vi "Test Assert Equal Value (Typedef).vi"(8 "error in":errorcluster) -> (0 "error out":errorcluster)   [LabVIEW 2020]
uses:
  <vilib>/Utility/error.llb/ErrWarn.ctl
  <vilib>/Utility/error.llb/DialogTypeEnum.ctl
  <vilib>/picture/picture.llb/imagedata.ctl
  <vilib>/Utility/miscctls.llb/LVBoundsTypeDef.ctl
  classes/Assert/Assert Equal Value_Variant.vi
  classes/Assert/Assert.lvclass
  classes/Test/Test.lvclass
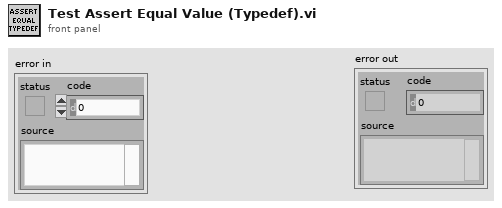
[diagram p1: front panel]
types:
  T1 = typedef "LVBoundsTypeDef.ctl" = cluster{"Width":u32, "Height":u32}
  T2 = cluster{"image type":i32, "image depth":i32, "image":u8[], "mask":u8[], "colors":u32[], "Rectangle":cluster{"left":i16, "top":i16, "right":i16, "bottom":i16}}
  T3 = typedef "imagedata.ctl" = cluster{"image type":i32, "image depth":i32, "image":u8[], "mask":u8[], "colors":u32[], "Rectangle":cluster{"left":i16, "top":i16, "right":i16, "bottom":i16}}
  T4 = enum16{"no dialog", "OK message", "continue or stop message", "auto error handling dialog", "OK message + warnings", "continue/stop + warnings"}
  T5 = typedef "DialogTypeEnum.ctl" = enum16{"no dialog", "OK message", "continue or stop message", "auto error handling dialog", "OK message + warnings", "continue/stop + warnings"}
  T6 = typedef "ErrWarn.ctl" = bool
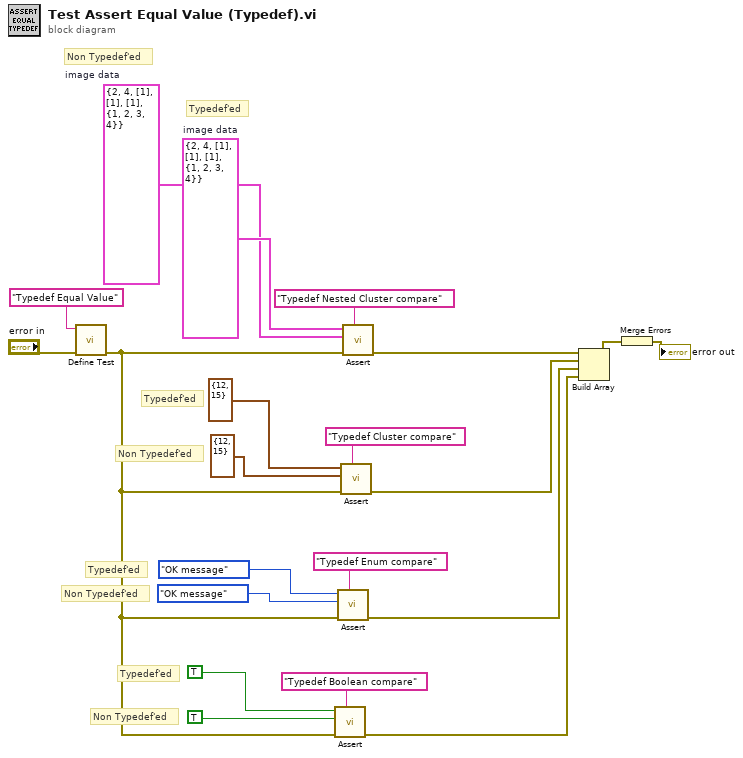
[diagram p0: block diagram]
diagram:
  w14 = T2 {"image type"=2, "image depth"=4, "image"=[1], "mask"=[1], "colors"=[1], "Rectangle"={"left"=1, "top"=2, "right"=3, "bottom"=4}}  # image data
  w15 = T3 {"image type"=2, "image depth"=4, "image"=[1], "mask"=[1], "colors"=[1], "Rectangle"={"left"=1, "top"=2, "right"=3, "bottom"=4}}  # image data
  # "Non Typedef'ed"
  # "Typedef'ed"
  # "Non Typedef'ed"
  # "Typedef'ed"
  # "Non Typedef'ed"
  # "Typedef'ed"
  # "Non Typedef'ed"
  # "Typedef'ed"
  n1 = call "Define Test.vi"("error in (no error)"="error in", "Label (VI Title)"="Typedef Equal Value" ("Label")) -> ("error out"=w5:errorcluster)  [unwired: 8 in, 1 out]
  n2 = call-poly "Assert.vi"("Label"="Typedef Boolean compare", "error in (no error)"=w5, "Y"=TRUE ("Boolean"), "X"=T6 TRUE ("Boolean")) -> ("error out"=w4:errorcluster)  [unwired: 6 in, 1 out]
  n3 = call-poly "Assert.vi"("Label"="Typedef Enum compare", "error in (no error)"=w5, "Y"=T4."OK message" ("type of dialog (OK msg:1)"), "X"=DialogTypeEnum."OK message" ("type of dialog (OK msg:1)")) -> ("error out"=w9:errorcluster)  [unwired: 6 in, 1 out]
  n4 = call-poly "Assert.vi"("Label"="Typedef Cluster compare", "error in (no error)"=w5, "Y"=cluster{"Width":u32, "Height":u32} {"Width"=12, "Height"=15} ("Bounds"), "X"=T1 {"Width"=12, "Height"=15} ("Bounds")) -> ("error out"=w10:errorcluster)  [unwired: 6 in, 1 out]
  n5 = call-poly "Assert.vi"("Label"="Typedef Nested Cluster compare", "error in (no error)"=w5, "Y"=w14, "X"=w15) -> ("error out"=w17:errorcluster)  [unwired: 6 in, 1 out]
  n6 = Build Array(w17, w10, w9, w4) -> (w19:errorcluster[])
  n7 = Merge Errors(w19) -> (→"error out":errorcluster)
